vi "Refresh Tag Exchange Prefix and Suffix.vi"(6 "Tag Exchange Tab References":T1, 8 "error in (no error)":errorcluster, 11 "E2E editor node in":refnum<data-value>) -> (0 "error out":errorcluster, 3 "E2E editor node out":refnum<data-value>)   [LabVIEW 2015, in "E2E Tag Exchange editor node.lvclass"]
uses:
  E2E Tag Exchange editor node.lvclass
  Tag Exchange Tab References.ctl
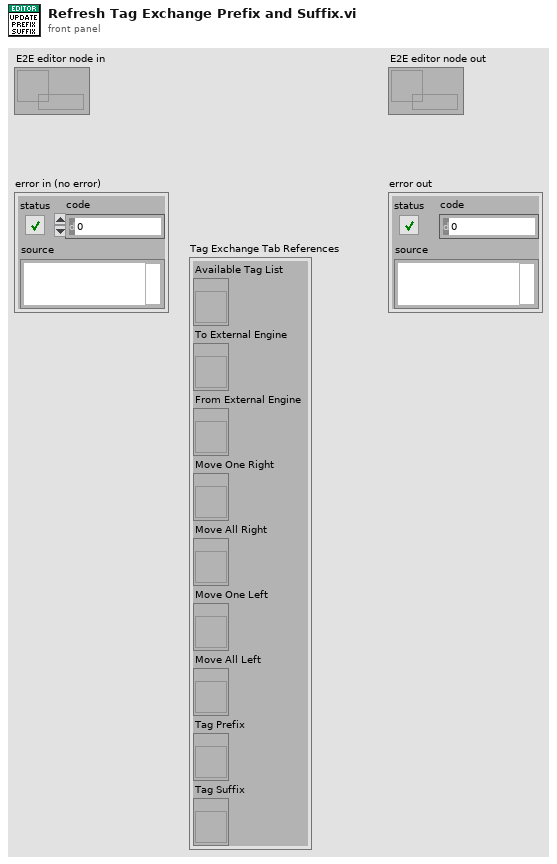
[diagram p1: front panel]
types:
  T1 = typedef "E2E Tag Exchange editor node.lvclass/Tag Exchange Tab References.ctl" = cluster{"Available Tag List":refnum<vi>, "To External Engine":refnum<vi>, "From External Engine":refnum<vi>, "Move One Right":refnum<vi>, "Move All Right":refnum<vi>, "Move One Left":refnum<vi>, "Move All Left":refnum<vi>, "Tag Prefix":refnum<vi>, "Tag Suffix":refnum<vi>}
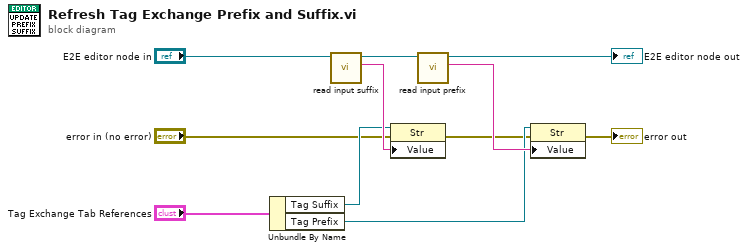
[diagram p0: block diagram]
diagram:
  n1 = Unbundle By Name("Tag Exchange Tab References") -> ("Tag Suffix"=w5:refnum<vi>, "Tag Prefix"=w4:refnum<vi>)
  n2 = call "read input suffix.vi"("E2E editor node in"="E2E editor node in") -> ("Input Suffix"=w9:string, "E2E editor node out"=w8:refnum<data-value>)  [unwired: 8 in, 1 out]
  n3 = property class="Str"(reference=w5, error in="error in (no error)", "Value"=w9) -> (error out=w1:errorcluster)  [unwired: 1 out]
  n4 = call "read input prefix.vi"("E2E editor node in"=w8) -> ("Input Prefix"=w10:string, "E2E editor node out"=→"E2E editor node out":refnum<data-value>)  [unwired: 8 in, 1 out]
  n5 = property class="Str"(reference=w4, error in=w1, "Value"=w10) -> (error out=→"error out":errorcluster)  [unwired: 1 out]
